vi "thermalCamera.vi"() -> ()   [LabVIEW 2025]
panel:
  out "Image":T1(plugin-control)
  out "IP address":string
  in  "Stop Button":bool
  out "Output":string
  in  "Flag":bool
  in  "Stop recording":bool
  in  "Stop Preview":bool
  in  "Server Path":path
  in  "Focus":dbl(slide) scale=0.0..100.0
  in  "Record":bool
  in  "Connect Server":bool
  out "?":string
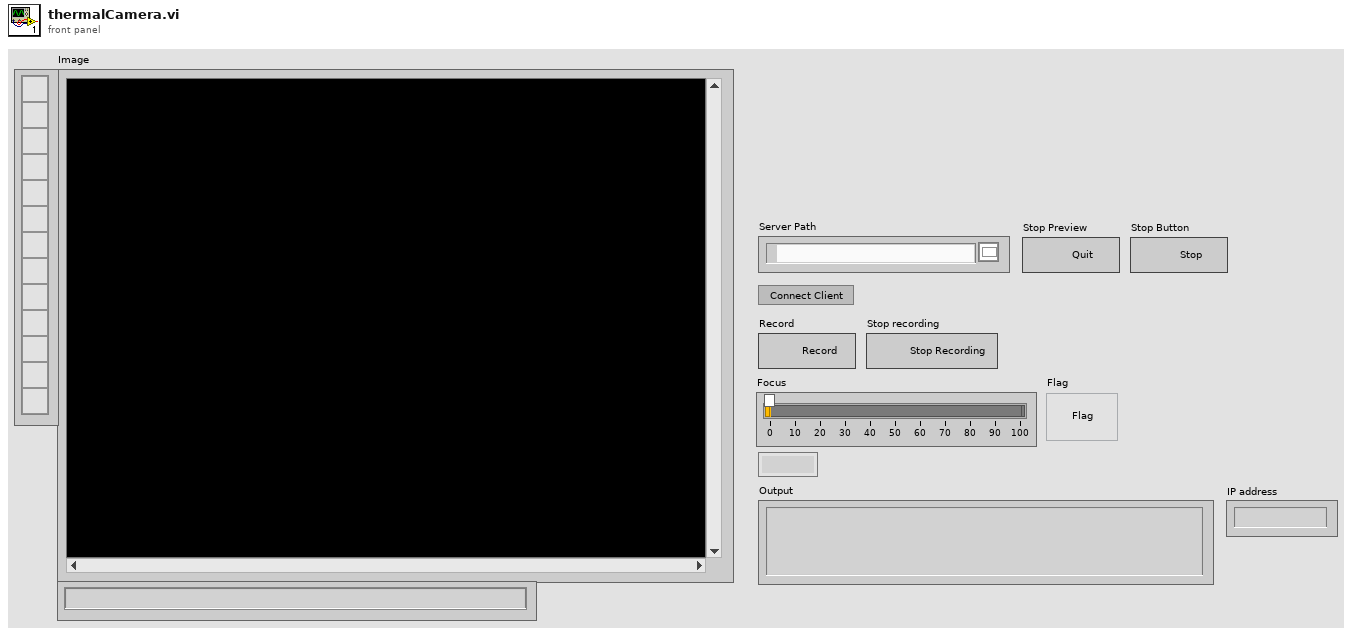
[diagram p1: front panel]
types:
  T1 = typedef "IMAQ Image.ctl" = refnum<image>
  T2 = typedef "Image Type" = u32
  T3 = enum16{"open", "replace", "create", "open or create", "replace or create", "replace or create with confirmation"}
  T4 = enum16{"big-endian, network order", "native, host order", "little-endian"}
  T5 = enum16{"Standard", "Buffered", "CRLF", "Immediate"}
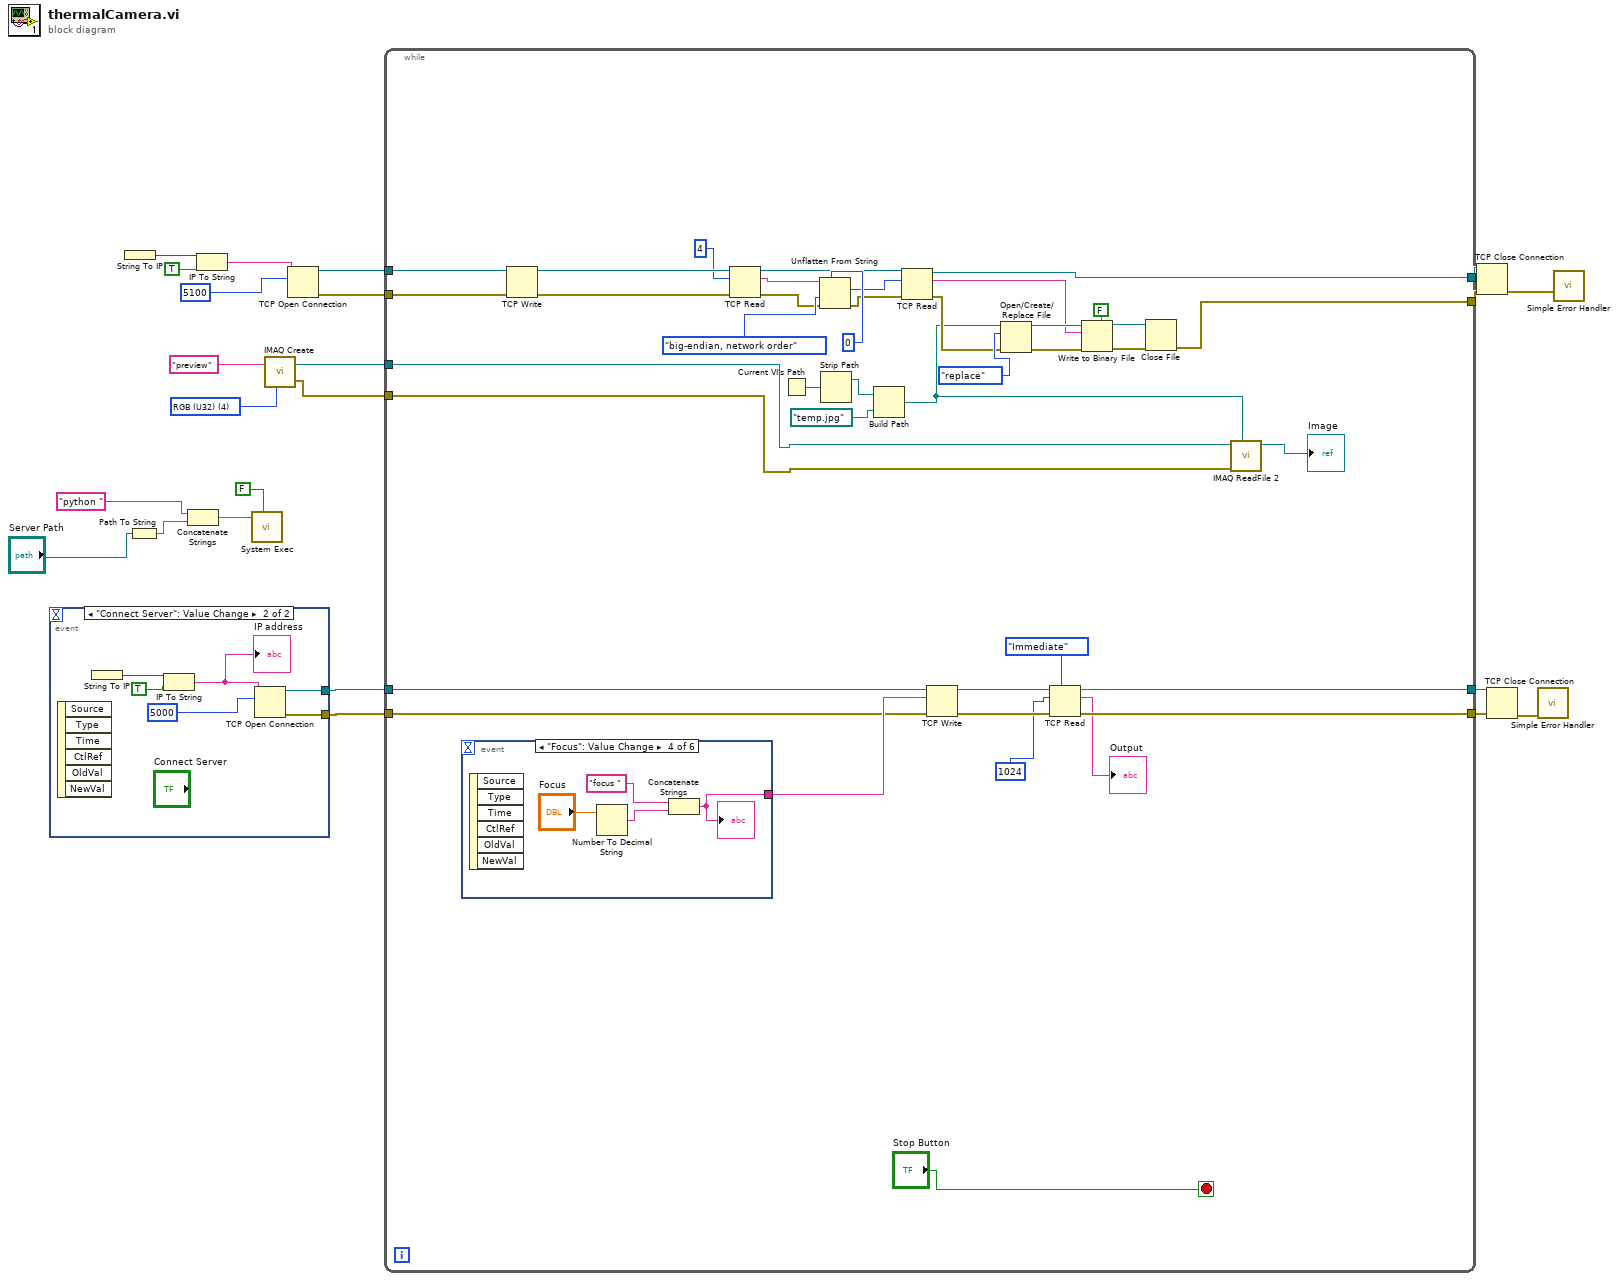
[diagram p0: block diagram]
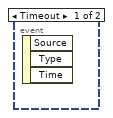
[diagram p2: hidden frame]
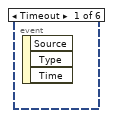
[diagram p3: hidden frame]
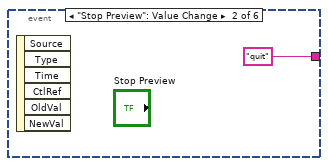
[diagram p4: hidden frame]
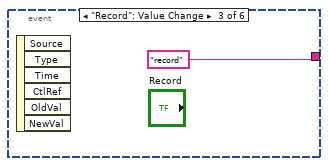
[diagram p5: hidden frame]
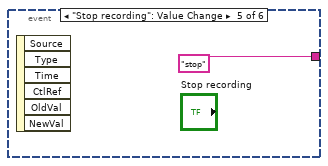
[diagram p6: hidden frame]
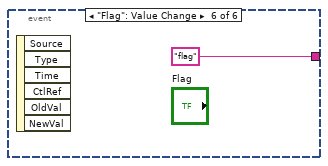
[diagram p7: hidden frame]
diagram:
  w3 = T2 4 items=["Grayscale (U8)", "Grayscale (I16)", "Grayscale (SGL)", "Complex (CSG)", "RGB (U32)", "HSL (U32)", "RGB (U64)", "Grayscale (U16)"] ("Image Type")
  n1 = event shown="[1] \"Connect Server\": Value Change" {
    selector: _ -> [_ _]
    dyn-events: _ -> [_ _]
    timeout: _ -> [_ _]
    tunnel: [_ w28] -> w18
    tunnel: [_ w27] -> w17
    event Timeout {
      n2 = event-data() -> ()  [unwired: 1 in, 3 out]
    }
    event "Connect Server": Value Change {
      n3 = event-data() -> ()  [unwired: 1 in, 6 out]
      n4 = String To IP() -> (0:w26:u32)  [unwired: 1 in]
      n5 = IP To String(1:TRUE ("dot notation? (F)"), 2:w26) -> (0:w24:string)
      "IP address" <- w24
      n6 = TCP Open Connection(address=w24, remote port or service name=u16 5000) -> (connection ID=w27:refnum<k5>, error out=w28:errorcluster)  [unwired: 3 in]
    }
  }
  n7 = String To IP() -> (0:w12:u32)  [unwired: 1 in]
  n8 = Path To String(path="Server Path") -> (string=w19:string)
  n9 = Concatenate Strings("python " ("string"), w19) -> (w15:string)
  n10 = IP To String(1:TRUE ("dot notation? (F)"), 2:w12) -> (0:w13:string)
  n11 = call <vilib>:"System Exec.vi"("wait until completion? (T)"=FALSE, "command line"=w15) -> ()  [unwired: 6 in, 4 out]
  n12 = call "IMAQ Create"("Image Name"="preview", "Image Type"=w3) -> ("New Image"=w2:T1, "error out"=w1:errorcluster)  [unwired: 3 in]
  n13 = TCP Open Connection(address=w13, remote port or service name=u16 5100) -> (connection ID=w9:refnum<k5>, error out=w8:errorcluster)  [unwired: 3 in]
  n14 = while {
    tunnel: [w68] -> w23
    tunnel: [w66] -> w22
    tunnel: w18 -> [w64]
    tunnel: w17 -> [w63]
    tunnel: w9 -> [w58]
    tunnel: w8 -> [w57]
    tunnel: [w34] -> w7
    tunnel: [w49] -> w6
    tunnel: w2 -> [w32]
    tunnel: w1 -> [w31]
    stop <- "Stop Button" stop-if-true
    n15 = event shown="[3] \"Focus\": Value Change" {
      selector: _ -> [_ _ _ _ _ _]
      dyn-events: _ -> [_ _ _ _ _ _]
      timeout: _ -> [_ _ _ _ _ _]
      tunnel: [_ "quit" "record" w73 "stop" "flag"] -> w65
      event Timeout {
        n16 = event-data() -> ()  [unwired: 1 in, 3 out]
      }
      event "Stop Preview": Value Change {
        n17 = event-data() -> ()  [unwired: 1 in, 6 out]
      }
      event "Record": Value Change {
        n18 = event-data() -> ()  [unwired: 1 in, 6 out]
      }
      event "Focus": Value Change {
        n19 = event-data() -> ()  [unwired: 1 in, 6 out]
        n20 = Number To Decimal String(number="Focus") -> (decimal integer string=w75:string)  [unwired: 1 in]
        n21 = Concatenate Strings("focus ", w75) -> (w73:string)
        "?" <- w73
      }
      event "Stop recording": Value Change {
        n22 = event-data() -> ()  [unwired: 1 in, 6 out]
      }
      event "Flag": Value Change {
        n23 = event-data() -> ()  [unwired: 1 in, 6 out]
      }
    }
    n24 = TCP Write(connection ID=w58, error in (no error)=w57) -> (connection ID out=w56:refnum<k5>, error out=w54:errorcluster)  [unwired: 2 in, 1 out]
    n25 = TCP Read(connection ID=w56, bytes to read=4, error in (no error)=w54) -> (connection ID out=w50:refnum<k5>, data out=w53:string, error out=w47:errorcluster)  [unwired: 2 in]
    n26 = Current VI's Path() -> (path=w45:path)
    n27 = Unflatten From String(type=0, binary string=w53, byte order (0:big-endian, network order)=T4."big-endian, network order", error in (no error)=w47) -> (value=w48:i32, error out=w46:errorcluster)  [unwired: 1 in, 1 out]
    n28 = Strip Path(path=w45) -> (stripped path=w44:path)  [unwired: 1 out]
    n29 = Build Path(base path=w44, name or relative path=path "temp.jpg") -> (appended path=w33:path)
    n30 = TCP Read(connection ID=w50, bytes to read=w48, error in (no error)=w46) -> (connection ID out=w49:refnum<k5>, data out=w40:string, error out=w37:errorcluster)  [unwired: 2 in]
    n31 = TCP Write(connection ID=w63, data in=w65, error in (no error)=w64) -> (connection ID out=w67:refnum<k5>, error out=w69:errorcluster)  [unwired: 1 in, 1 out]
    n32 = Open/Create/Replace File(file path (use dialog)=w33, error in=w37, operation (0:open)=T3."replace") -> (refnum out=w41:refnum<file>, error out=w36:errorcluster)  [unwired: 3 in, 1 out]
    n33 = TCP Read(connection ID=w67, bytes to read=1024, error in (no error)=w69, 7:T5."Immediate" ("mode (standard)")) -> (connection ID out=w66:refnum<k5>, data out=→"Output":string, error out=w68:errorcluster)  [unwired: 1 in]
    n34 = Write to Binary File(file (use dialog)=w41, data=w40, error in=w36, 5:FALSE ("prepend array or string size? (T)")) -> (refnum out=w38:refnum<file>, error out=w35:errorcluster)  [unwired: 2 in, 1 out]
    n35 = Close File(refnum=w38, error in=w35) -> (error out=w34:errorcluster)  [unwired: 1 out]
    n36 = call "IMAQ ReadFile 2"("File Path"=w33, "error in (no error)"=w31, "Image"=w32) -> ("Image Out"=→"Image":T1)  [unwired: 4 in, 4 out]
  }
  n37 = TCP Close Connection(connection ID=w6, error in (no error)=w7) -> (error out=w5:errorcluster)  [unwired: 1 in, 1 out]
  n38 = TCP Close Connection(connection ID=w22, error in (no error)=w23) -> (error out=w21:errorcluster)  [unwired: 1 in, 1 out]
  n39 = call <vilib>:"Simple Error Handler.vi"("error in (no error)"=w21) -> ()  [unwired: 4 in, 5 out]
  n40 = call <vilib>:"Simple Error Handler.vi"("error in (no error)"=w5) -> ()  [unwired: 4 in, 5 out]
